vi "Watchdog Set Attribute.vi"(4 "attribute":T1, 5 "error in (no error)":errorcluster, 7 "attribute value":u32, 8 "watchdogID in":u64=1 format="%.0x") -> (0 "error out":errorcluster, 2 "attribute value returned":u32, 3 "watchdogID out":u64=1 format="%.0x")   [LabVIEW 2025]
doc: "<p>Sets the <a href=\"nihelplauncher://docs/csh?context=lvrt_lvrtconcepts_rt_watchdog\">watchdog object</a> attribute you specify to the value you specify.</p>"
uses:
  niwd4c.dll
  Watchdog attribute enum.ctl
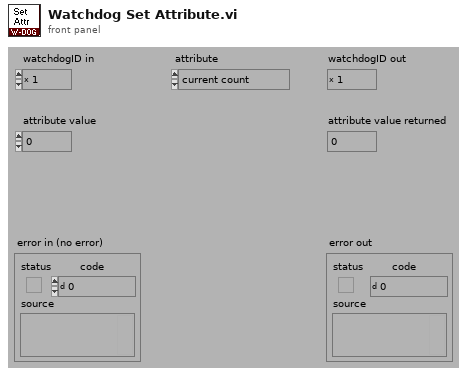
[diagram p1: front panel]
types:
  T1 = typedef "Watchdog attribute enum.ctl" = enum16{"current count", "hardware expire", "hardware ID", "hardware lock", "initial count", "instance", "resolution", "time step", "whack input source", "total timeout"}
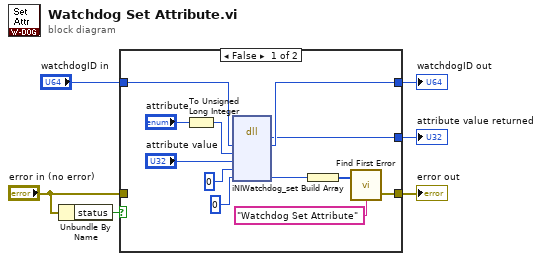
[diagram p0: block diagram]
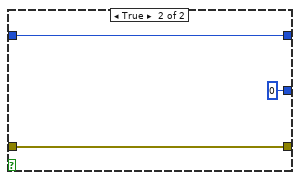
[diagram p2: hidden frame]
diagram:
  n1 = Unbundle By Name("error in (no error)") -> ("status"=w1:bool)
  n2 = case shown="False" w1 {
    tunnel: [w11 w20] -> w4
    tunnel: [w17 w21] -> w3
    tunnel: "error in (no error)" -> [_ w21]
    tunnel: "watchdogID in" -> [w14 w20]
    tunnel: [w8 0 ("value")] -> w2
    frame False {
      n3 = To Unsigned Long Integer(number="attribute") -> (unsigned 32bit integer=w13:u32)
      n4 = dll-call lib="niwd4c.*" fn="iNIWatchdog_set" label="Set"("wd"=w14, "attribute"=w13, "value"="attribute value", "timeUnit"=u32 0, "status"=0) -> ("return type"=w8:u32, "wd"=w11:u64, "status"=w9:i32)  [unwired: 6 in, 2 out]
      n5 = Build Array(w9) -> (w18:i32[])
      n6 = call <vilib>:"Find First Error.vi"("source messages"="Watchdog Set Attribute", "error codes"=w18) -> ("error out"=w17:errorcluster)  [unwired: 2 in, 1 out]
    }
    frame True {
    }
  }
  "error out" <- w3
  "watchdogID out" <- w4
  "attribute value returned" <- w2
